vi "Scale Setting Description.vi"(11 "Sacle Setting Out":T1) -> (3 "Description":string)   [LabVIEW 2020, in "Data Viewer.lvlib" / "Data Viewer.lvclass"]
uses:
  Data Viewer.lvclass
  Scale Setting--cluster.ctl
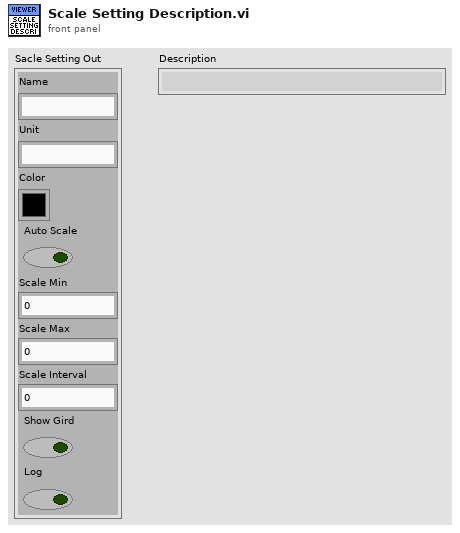
[diagram p1: front panel]
types:
  T1 = typedef "Data Viewer.lvlib/Data Viewer.lvclass/Scale Setting--cluster.ctl" = cluster{"Name":string, "Unit":string, "Color":u32, "Auto Scale":bool, "Scale Min":dbl, "Scale Max":dbl, "Scale Interval":dbl, "Show Gird":bool, "Log":bool}
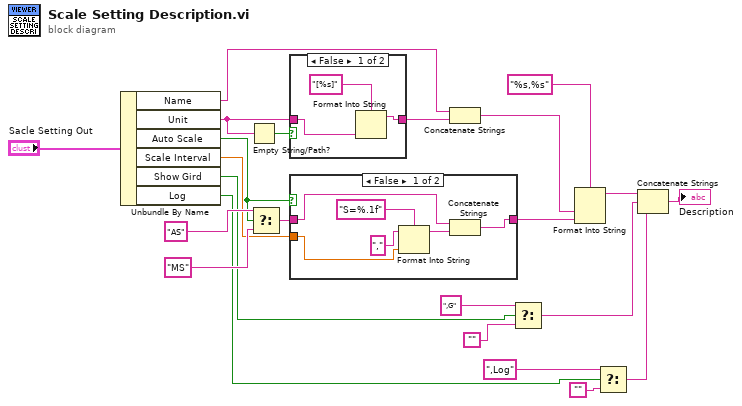
[diagram p0: block diagram]
diagram:
  n1 = Unbundle By Name("Sacle Setting Out") -> ("Name"=w20:string, "Unit"=w21:string, "Auto Scale"=w16:bool, "Scale Interval"=w14:dbl, "Show Gird"=w13:bool, "Log"=w10:bool)
  n2 = Empty String/Path?(string/path=w21) -> (empty?=w22:bool)
  n3 = Select(t="AS", s=w16, f="MS") -> (s? t:f=w15:string)
  n4 = case shown="False" w22 {
    tunnel: w21 -> [w26 w27]
    tunnel: [w24 w27] -> w19
    frame False {
      n5 = Format Into String(format string="[%s]", w26) -> (resulting string=w24:string)  [unwired: 2 in, 1 out]
    }
    frame True {
    }
  }
  n6 = case shown="False" w16 {
    tunnel: [w28 w34] -> w8
    tunnel: w15 -> [w29 w34]
    tunnel: w14 -> [w33 _]
    frame False {
      n7 = Format Into String(format string="S=%.1f", initial string=",", w33) -> (resulting string=w30:string)  [unwired: 1 in, 1 out]
      n8 = Concatenate Strings(w29, w30) -> (w28:string)
    }
    frame True {
    }
  }
  n9 = Concatenate Strings(w20, w19) -> (w9:string)
  n10 = Select(t=",G", s=w13, f="") -> (s? t:f=w2:string)
  n11 = Format Into String(format string="%s,%s", w9, w8) -> (resulting string=w5:string)  [unwired: 2 in, 1 out]
  n12 = Select(t=",Log", s=w10, f="") -> (s? t:f=w1:string)
  n13 = Concatenate Strings(w5, w2, w1) -> (→"Description":string)
